vi "Create Waveform and Preview.vi"(5 "XYGraph Refnum":refnum<vi>, 7 "Program":T3(array[cluster]), 8 "error in (no error)":errorcluster, 10 "Waveform In":T1, 11 "Display State In":T2 caption="State" {"# of Loops" min=1 step=1; "Index" min=0 step=1; "Program"."Step" min=0.001 max=80.0 step=0.001 format="%.2f"; "Program"."Target" format="%.2f"}) -> (0 "error out":errorcluster, 1 "Preview Graph":cluster{dbl[], dbl[]}[](graph), 2 "Waveform Out":T1, 3 "State Out":T2 caption="State" {"# of Loops" min=1 step=1; "Index" min=0 step=1; "Program"."Step" min=0.001 max=80.0 step=0.001 format="%.2f"; "Program"."Target" format="%.2f"})   [LabVIEW 2012, in "Multi Segment Waveform.xctl"]
doc: "Build Preview with current marker and y=0 line"
uses:
  Multi Segment Waveform.xctl
  State.ctl
  Data.ctl
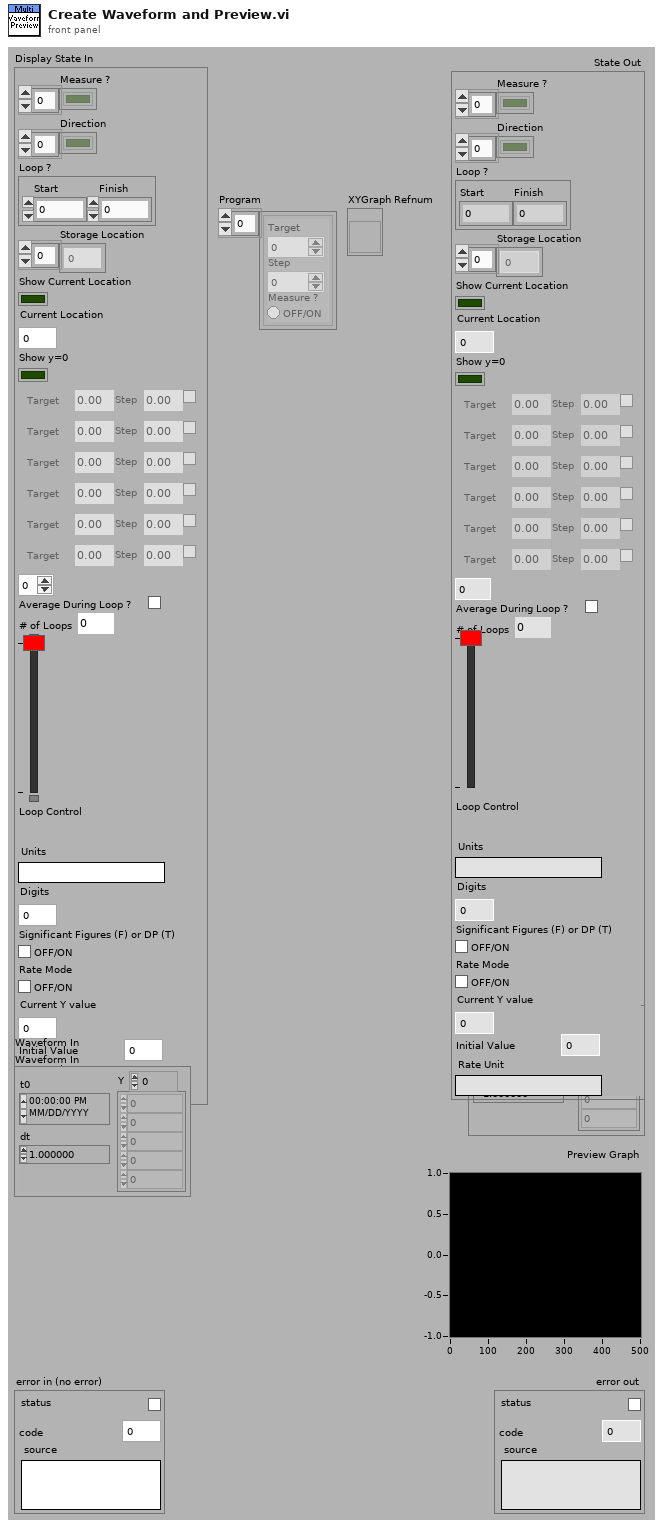
[diagram p1: front panel]
types:
  T1 = typedef "Multi Segment Waveform.xctl/Data.ctl" = waveform(dbl)
  T2 = typedef "Multi Segment Waveform.xctl/State.ctl" = cluster{"Measure ?":bool[], "Direction":bool[], "Loop ?":cluster{"Start":i32, "Finish":i32}, "Storage Location":i32[], "Show Current Location":bool, "Current Location":i32, "Show y=0":bool, "Program":cluster{"Target":dbl, "Step":dbl, "Measure ?":bool}[], "Index":i32, "Average During Loop ?":bool, "# of Loops":u32, "Loop Control":cluster{i32, i32}, "Units":string, "Digits":i32, "Significant Figures (F) or DP (T)":bool, "Rate Mode":bool, "Current Y value":dbl, "Initial Value":dbl, "Rate Unit":string}
  T3 = cluster{"Target":dbl, "Step":dbl, "Measure ?":bool}[]
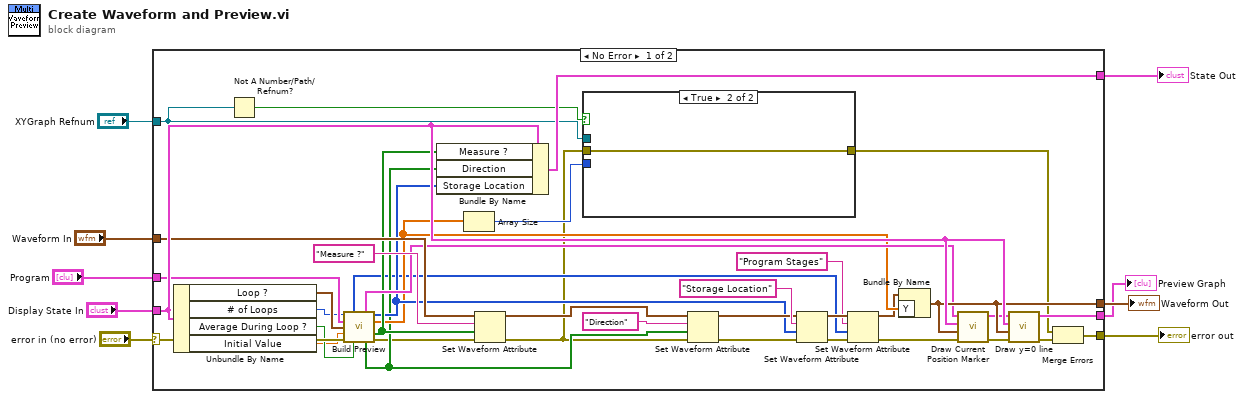
[diagram p0: block diagram]
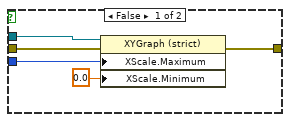
[diagram p2: hidden frame]
diagram:
  n1 = case shown="No Error" "error in (no error)" {
    selector: "error in (no error)" -> [w25 w55]
    tunnel: "Display State In" -> [w47 w54]
    tunnel: [w45 _] -> w8
    tunnel: [w44 _] -> w7
    tunnel: "Program" -> [w37 _]
    tunnel: [w36 w54] -> w5
    tunnel: "Waveform In" -> [w35 _]
    tunnel: "XYGraph Refnum" -> [w15 _]
    tunnel: [w13 w55] -> w1
    frame No Error {
      n2 = Unbundle By Name(w47) -> ("Loop ?"=w34:cluster{"Start":i32, "Finish":i32}, "# of Loops"=w17:u32, "Average During Loop ?"=w16:bool, "Initial Value"=w10:dbl)
      n3 = Not A Number/Path/Refnum?(number/path/refnum=w15) -> (NaN/Path/Refnum?=w11:bool)
      n4 = call "Build Preview.vi"("# Of Loops"=w17, "Program"=w37, "Loop ?"=w34, "Initial Value"=w10, "error in (no error)"=w25, "Average During Loop ?"=w16) -> ("Stage Values"=w21:i32[], "Plots Out"=w33:cluster{dbl[], dbl[]}[], "Storage Locations Out"=w31:i32[], "Y Values Out"=w30:dbl[], "Measure ? Out"=w32:bool[], "Direction Out"=w27:bool[], "error out"=w26:errorcluster)  [unwired: 3 in]
      n5 = Bundle By Name(cluster=w47, "Measure ?"=w32, "Direction"=w27, "Storage Location"=w31) -> (w36:T2)
      n6 = Array Size(array=w30) -> (size(s)=w46:i32)
      n7 = Set Waveform Attribute(4:w26, 5:w32, 6:"Measure ?" ("name"), 7:w35) -> (0:w14:errorcluster, 3:w38:T1)  [unwired: 1 out]
      n8 = case shown="True" w11 {
        tunnel: w46 -> [w51 _]
        tunnel: w15 -> [w50 _]
        tunnel: w14 -> [w49 w53]
        tunnel: [w48 w53] -> w12
        frame False {
          n9 = property on="Property Node" class="XYGraph (strict)"(reference=w50, error in=w49, "XScale.Maximum"=w51, "XScale.Minimum"=0.0 ("X Scale.Range:Minimum")) -> (error out=w48:errorcluster)  [unwired: 1 out]
        }
        frame True {
        }
      }
      n10 = Set Waveform Attribute(4:w14, 5:w27, 6:"Direction" ("name"), 7:w38) -> (0:w28:errorcluster, 3:w39:T1)  [unwired: 1 out]
      n11 = Set Waveform Attribute(4:w28, 5:w31, 6:"Storage Location" ("name"), 7:w39) -> (0:w23:errorcluster, 3:w22:T1)  [unwired: 1 out]
      n12 = Set Waveform Attribute(4:w23, 5:w21, 6:"Program Stages" ("name"), 7:w22) -> (0:w18:errorcluster, 3:w19:T1)  [unwired: 1 out]
      n13 = Bundle By Name(cluster=w19, "Y"=w30) -> (w45:T1)
      n14 = call "Draw Current Position Marker.vi"("Error"=w18, "Waveform"=w45, "State"=w47, "Plots"=w33) -> ("Error Out"=w29:errorcluster, "Plots Out"=w43:cluster{"X":dbl[], "Y":dbl[]}[])  [unwired: 6 out]
      n15 = call "Draw y=0 line.vi"("Error"=w29, "Waveform"=w45, "State"=w47, "Plots"=w43) -> ("Error Out"=w24:errorcluster, "Plots Out"=w44:cluster{"X":dbl[], "Y":dbl[]}[])  [unwired: 6 out]
      n16 = Merge Errors(w12, w24) -> (w13:errorcluster)
    }
    frame Error {
    }
  }
  "Preview Graph" <- w7
  "Waveform Out" <- w8
  "State Out" <- w5
  "error out" <- w1
